vi "Member.vi"(8 "error in (no error)":errorcluster, 11 "FixtureClass in":refnum<class "FixtureClass.lvclass">) -> (0 "error out":errorcluster, 3 "FixtureClass out":refnum<class "FixtureClass.lvclass">)   [LabVIEW 2024, in "FixtureClass.lvclass"]
doc: "Passes the FixtureClass instance through unchanged."
uses:
  FixtureClass.lvclass
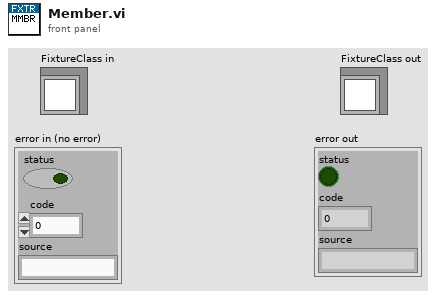
[diagram p1: front panel]
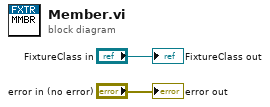
[diagram p0: block diagram]
diagram:
  "FixtureClass out" <- "FixtureClass in"
  "error out" <- "error in (no error)"
